vi "Create Stub Files.vi"(8 "error in":errorcluster, 11 "Main Destination Path":path) -> (0 "error out":errorcluster, 3 "Main Destination Path Out":path)   [LabVIEW 2027, in "Build VIs.lvlib"]
uses:
  Build VIs.lvlib
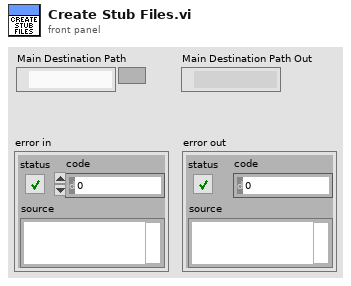
[diagram p1: front panel]
types:
  T1 = enum16{"open", "replace", "create", "open or create", "replace or create", "replace or create with confirmation"}
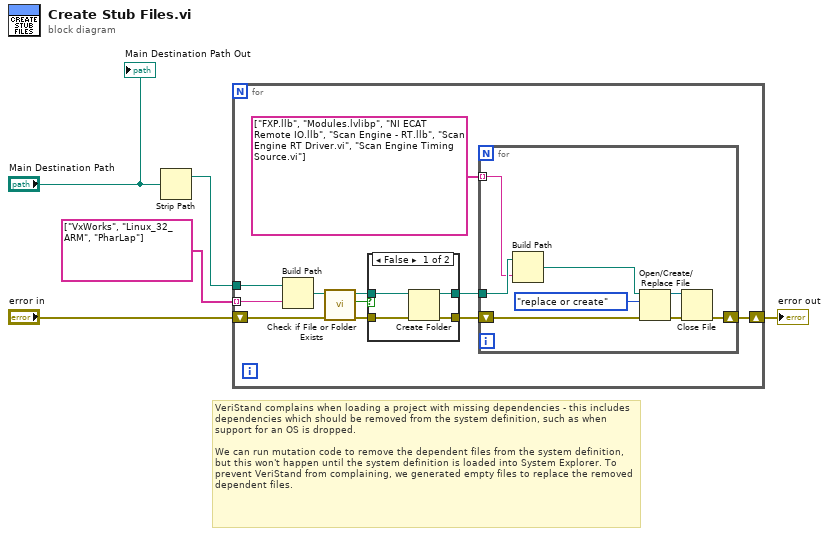
[diagram p0: block diagram]
diagram:
  # "VeriStand complains when loading a project with missing dependencies - this includes dependencies which should be removed from the system definition, such as when support for an OS is dropped.\n\nWe can run mutation code to remove the dependent files from the system definition, but this won't happen until the system definition is loaded into System Explorer. To prevent VeriStand from complaining, we generated empty files to replace the removed dependent files."
  n1 = Strip Path(path="Main Destination Path") -> (stripped path=w4:path)  [unwired: 1 out]
  n2 = for {
    tunnel: w4 -> [w16]
    tunnel: string[] ["VxWorks", "Linux_32_ARM", "PharLap"] -> [w15] mode=indexing
    shift-right: [w11] -> w3
    shift-left: "error in" -> [w8]
    n3 = Build Path(base path=w16, name or relative path=w15) -> (appended path=w10:path)
    n4 = call <vilib>:"Check if File or Folder Exists.vi"("error in (no error)"=w8, "path"=w10) -> ("error out"=w7:errorcluster, "file or folder exists?"=w6:bool, "dup path"=w9:path)  [unwired: 7 in]
    n5 = case shown="False" w6 {
      tunnel: [w20 w22] -> w13
      tunnel: [w19 w21] -> w12
      tunnel: w9 -> [w18 w22]
      tunnel: w7 -> [w17 w21]
      frame False {
        n6 = Create Folder(path (use dialog)=w18, error in=w17) -> (created path=w20:path, error out=w19:errorcluster)  [unwired: 1 in, 1 out]
      }
      frame True {
      }
    }
    n7 = for {
      tunnel: w13 -> [w30]
      tunnel: string[] ["FXP.llb", "Modules.lvlibp", "NI ECAT Remote IO.llb", "Scan Engine - RT.llb", "Scan Engine RT Driver.vi", "Scan Engine Timing Source.vi"] ("name or relative path") -> [w29] mode=indexing
      shift-right: [w24] -> w11
      shift-left: w12 -> [w27]
      n8 = Build Path(base path=w30, name or relative path=w29) -> (appended path=w28:path)
      n9 = Open/Create/Replace File(file path (use dialog)=w28, error in=w27, operation (0:open)=T1."replace or create") -> (refnum out=w23:refnum<file>, error out=w26:errorcluster)  [unwired: 3 in, 1 out]
      n10 = Close File(refnum=w23, error in=w26) -> (error out=w24:errorcluster)  [unwired: 1 out]
    }
  }
  "error out" <- w3
  "Main Destination Path Out" <- "Main Destination Path"
